vi "UI_Render_Main.vi"(0 "Channels":T1(array[cluster]), 1 "Logging":bool, 2 "Hover Button":i32=-1, 3 "Phase":bool, 5 "Data":dbl[][](array[numeric]), 7 "dt":dbl=0.001, 9 "Running":bool, 11 "error in":errorcluster, 12 "Status":string) -> (4 "Picture":picture, 15 "error out":errorcluster)   [LabVIEW 2026]
doc: "메인 화면 1600x940 전체 그리기: 주황 제목 띠 + 버튼 6개, 128채널 타일 바둑판, 하단 그래프 카드."
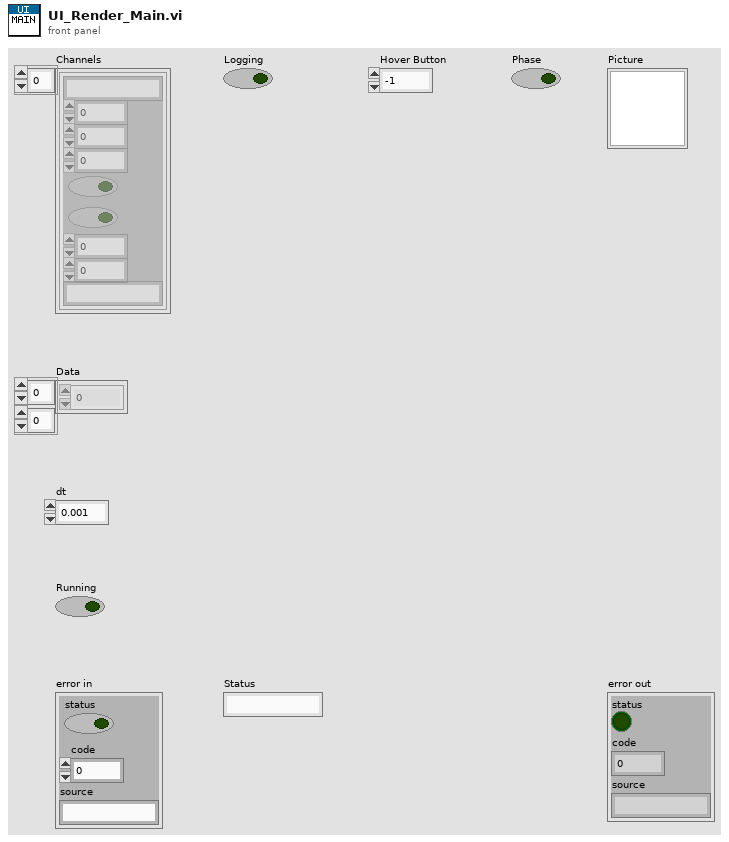
[diagram p1: front panel]
types:
  T1 = cluster{"Name":string, "Value":dbl, "High Limit":dbl, "Low Limit":dbl, "Save":bool, "Graph":bool, "Scale Min":dbl, "Scale Max":dbl, "Unit":string}[]
  T2 = cluster{"left":i16, "top":i16, "right":i16, "bottom":i16}
  T3 = cluster{"Font Name:":string, "Size":i16, "Strikeout?":bool, "Italic?":bool, "Underline?":bool, "Outline?":bool, "Shadow?":bool, "Bold?":bool}
  T4 = enum16{"User-specified Font", "Application Font", "System Font", "Dialog Font"}
  T5 = cluster{"horizontal":enum16{"left", "center", "right"}, "vertical":enum16{"top", "center", "bottom"}}
  T6 = cluster{"Width":u16, "Style":enum32{"Solid", "Dash", "Dot", "DashDot", "DashDotDot"}}
  T7 = cluster{"Rect":cluster{"left":i16, "top":i16, "right":i16, "bottom":i16}, "Fill":u32, "Fill Sel":u32, "Border":u32, "Border Sel":u32, "Text":string, "Text Color":u32, "Text Sel":u32, "Size":i16, "Bold":bool, "Group":i32, "Value":i32, "Radius":i16}[]
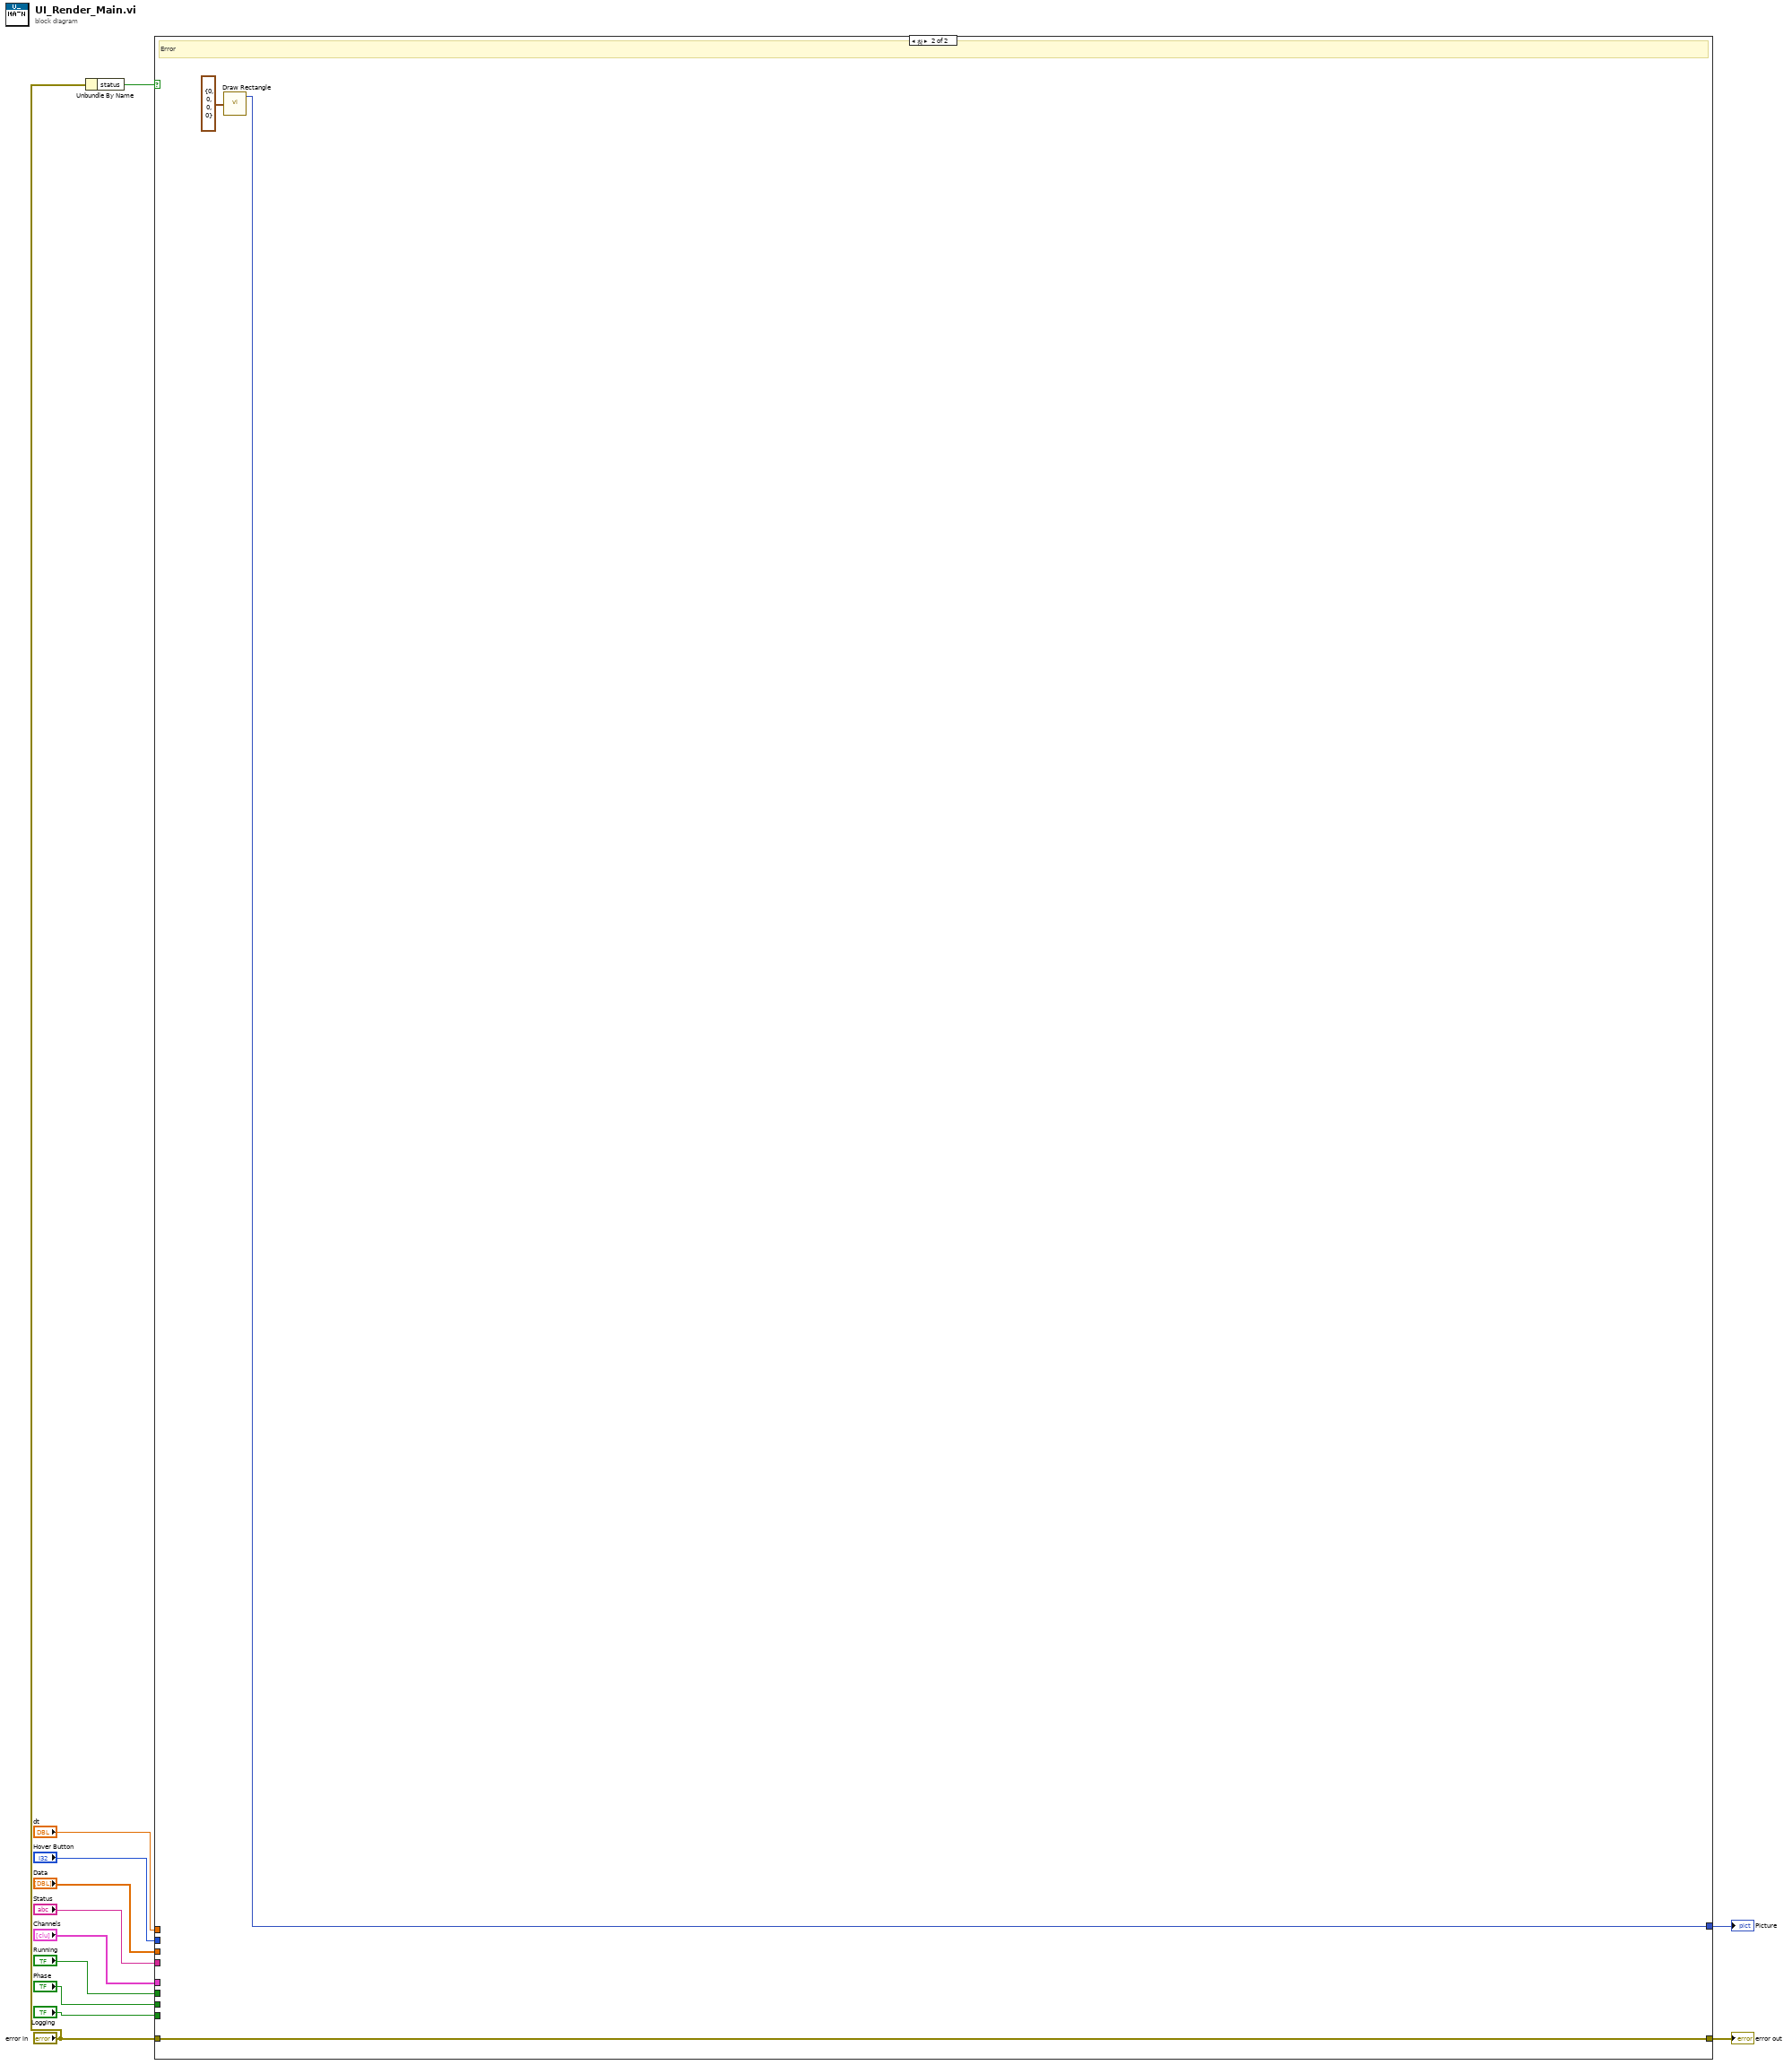
[diagram p0: block diagram]
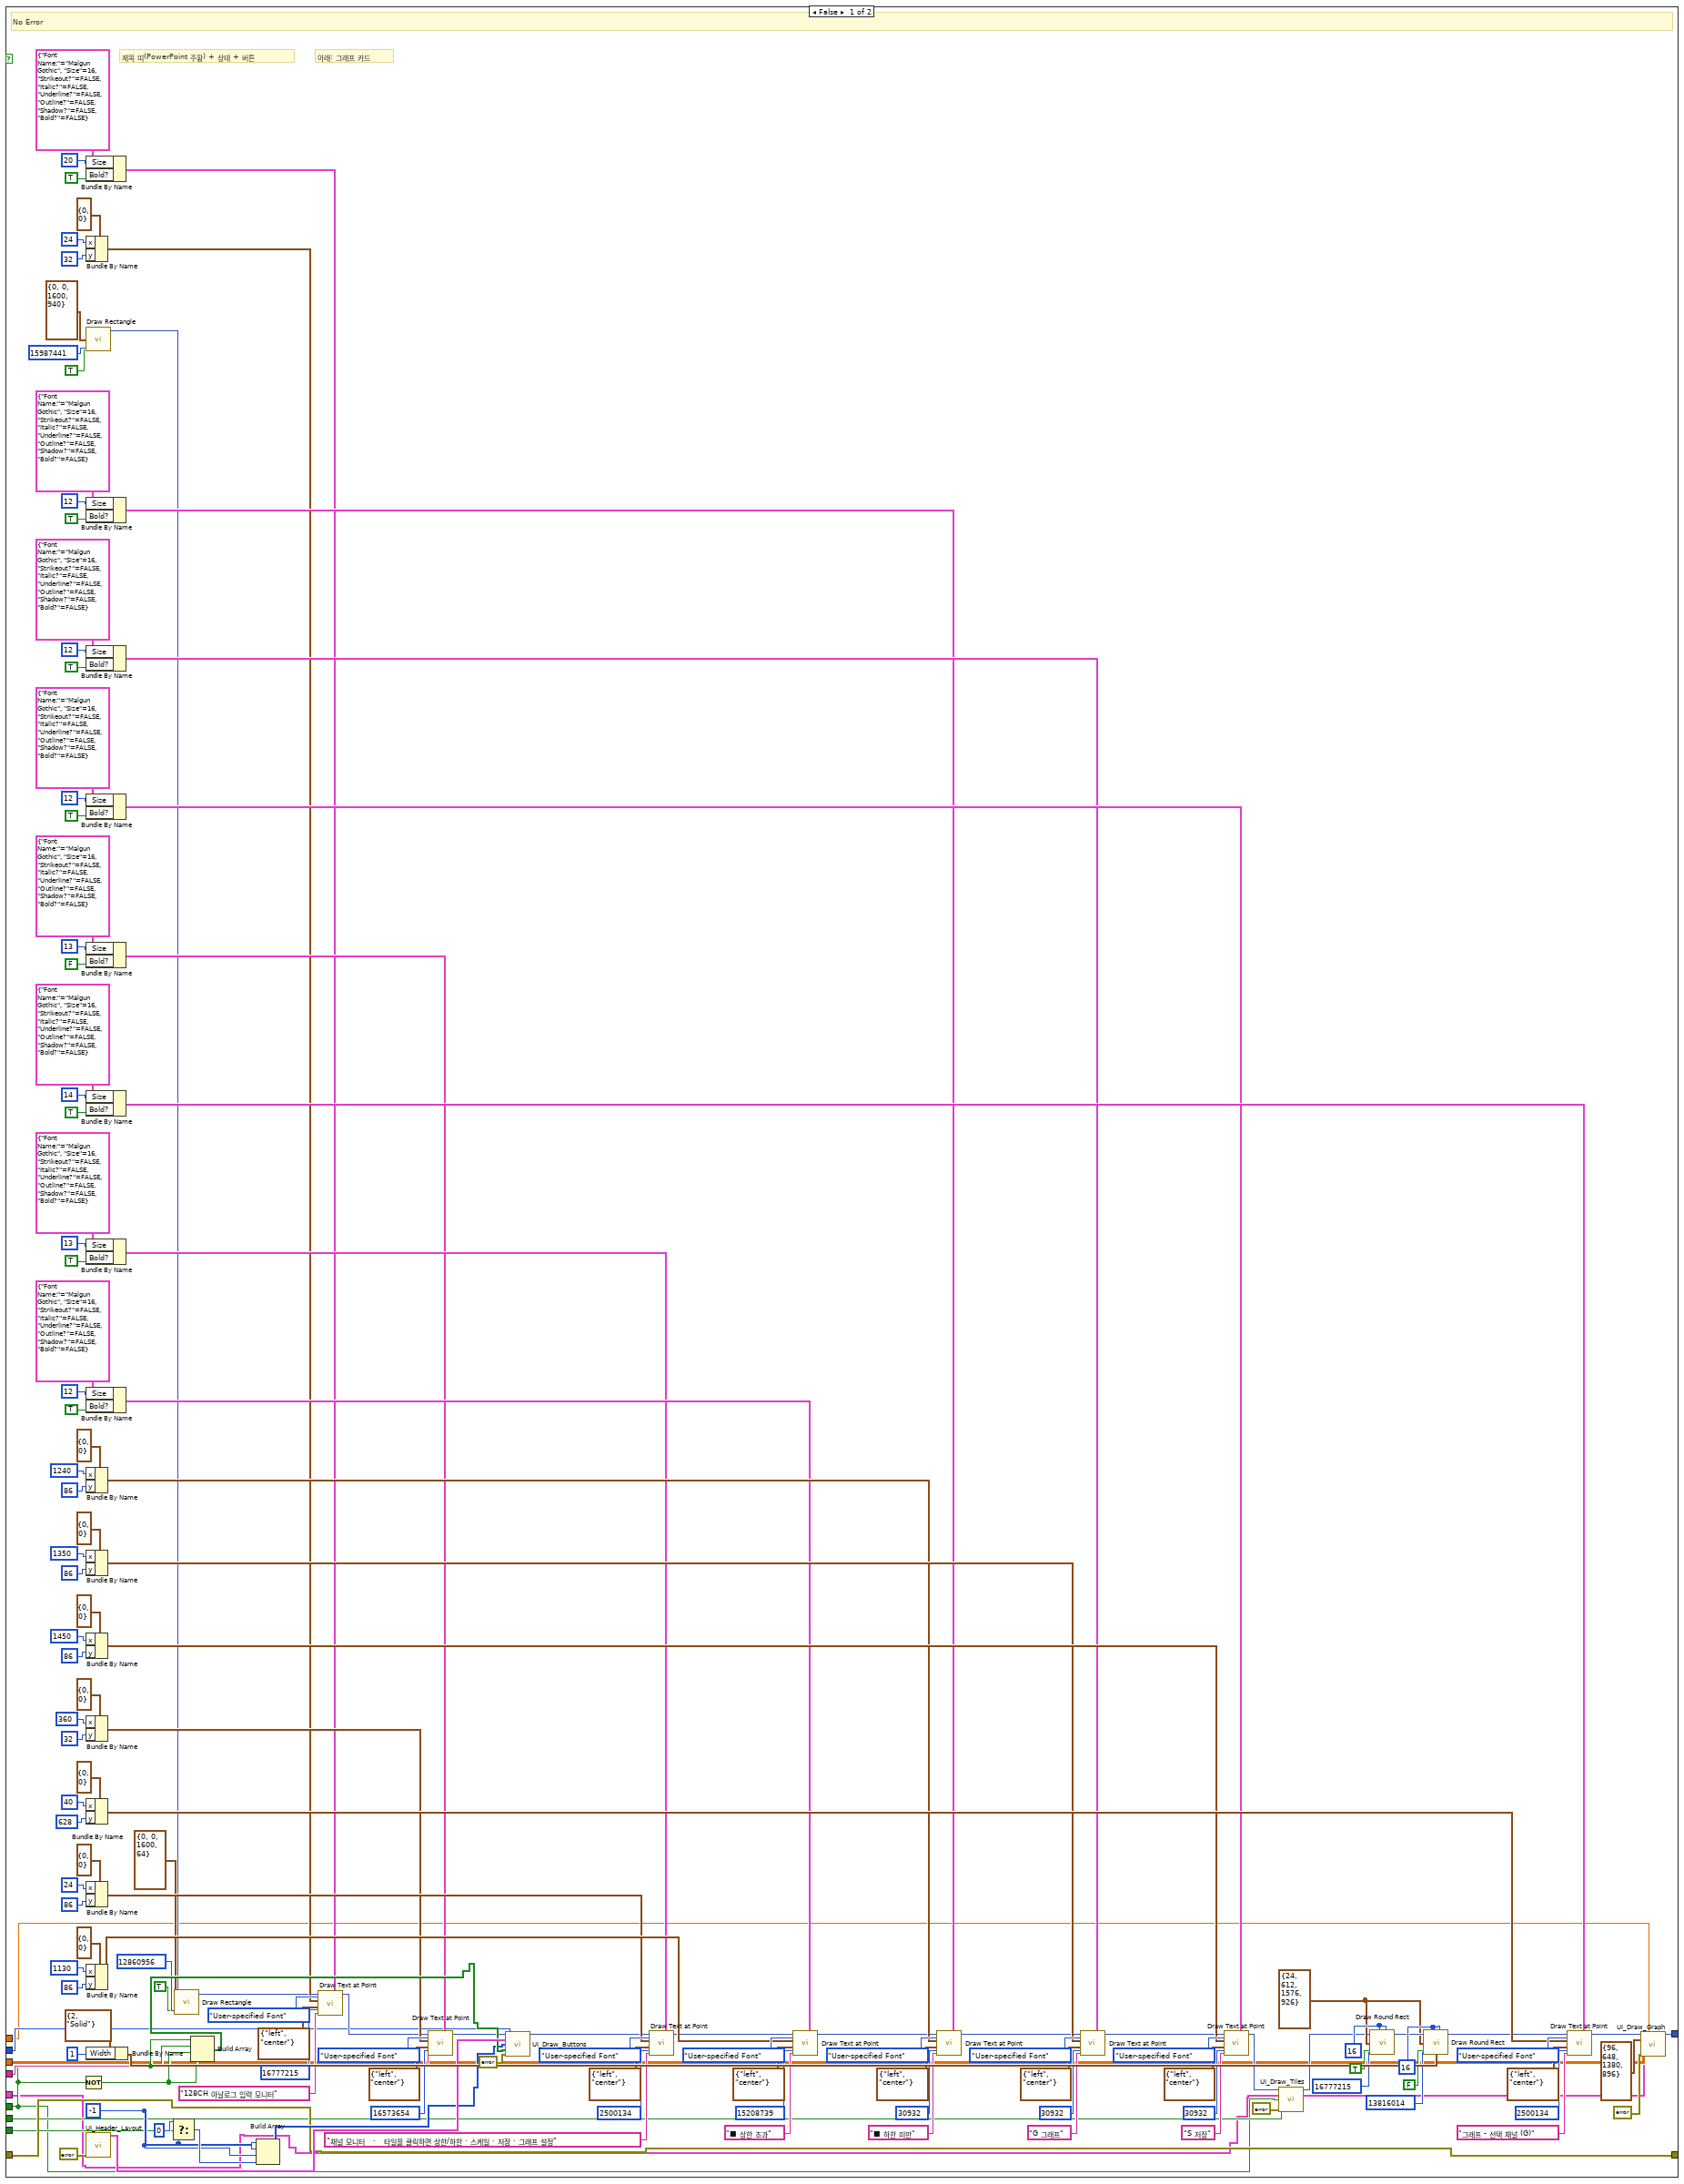
[diagram p2: hidden frame]
diagram:
  n1 = Unbundle By Name("error in") -> ("status"=w10:bool)
  n2 = case shown="참" w10 {
    tunnel: "Channels" -> [w13 _]
    tunnel: "Data" -> [w14 _]
    tunnel: "dt" -> [w15 _]
    tunnel: "Running" -> [w16 _]
    tunnel: "Logging" -> [w17 _]
    tunnel: "Hover Button" -> [w18 _]
    tunnel: "Phase" -> [w19 _]
    tunnel: "Status" -> [w20 _]
    tunnel: "error in" -> [w21 w160]
    tunnel: [w21 w160] -> w12
    tunnel: [w159 w162] -> w11
    frame False {
      w138 = i16 16
      w134 = i16 16
      w132 = T2 {"left"=24, "top"=612, "right"=1576, "bottom"=926}
      w55 = -1
      # "아래: 그래프 카드"
      # "제목 띠(PowerPoint 주황) + 상태 + 버튼"
      # "No Error"
      n3 = Not(x=w16) -> (.not. x?=w59:bool)
      n4 = Bundle By Name(cluster=T3 {"Font Name:"="Malgun Gothic", "Size"=16, "Strikeout?"=FALSE, "Italic?"=FALSE, "Underline?"=FALSE, "Outline?"=FALSE, "Shadow?"=FALSE, "Bold?"=FALSE}, "Size"=i16 20, "Bold?"=TRUE) -> (w41:T3)
      n5 = Bundle By Name(cluster=cluster{"x":i16, "y":i16} {"x"=0, "y"=0}, "x"=i16 24, "y"=i16 32) -> (w37:cluster{"x":i16, "y":i16})
      n6 = call <vilib>:"Draw Rectangle.vi"("rect"=T2 {"left"=0, "top"=0, "right"=1600, "bottom"=940}, "fill?(F)"=TRUE, "color(black)"=u32 15987441) -> ("new picture"=w25:picture)  [unwired: 6 in]
      n7 = Bundle By Name(cluster=T3 {"Font Name:"="Malgun Gothic", "Size"=16, "Strikeout?"=FALSE, "Italic?"=FALSE, "Underline?"=FALSE, "Outline?"=FALSE, "Shadow?"=FALSE, "Bold?"=FALSE}, "Size"=i16 12, "Bold?"=TRUE) -> (w102:T3)
      n8 = Bundle By Name(cluster=T3 {"Font Name:"="Malgun Gothic", "Size"=16, "Strikeout?"=FALSE, "Italic?"=FALSE, "Underline?"=FALSE, "Outline?"=FALSE, "Shadow?"=FALSE, "Bold?"=FALSE}, "Size"=i16 12, "Bold?"=TRUE) -> (w115:T3)
      n9 = Bundle By Name(cluster=T3 {"Font Name:"="Malgun Gothic", "Size"=16, "Strikeout?"=FALSE, "Italic?"=FALSE, "Underline?"=FALSE, "Outline?"=FALSE, "Shadow?"=FALSE, "Bold?"=FALSE}, "Size"=i16 12, "Bold?"=TRUE) -> (w128:T3)
      n10 = Bundle By Name(cluster=T3 {"Font Name:"="Malgun Gothic", "Size"=16, "Strikeout?"=FALSE, "Italic?"=FALSE, "Underline?"=FALSE, "Outline?"=FALSE, "Shadow?"=FALSE, "Bold?"=FALSE}, "Size"=i16 13, "Bold?"=FALSE) -> (w53:T3)
      n11 = Bundle By Name(cluster=T3 {"Font Name:"="Malgun Gothic", "Size"=16, "Strikeout?"=FALSE, "Italic?"=FALSE, "Underline?"=FALSE, "Outline?"=FALSE, "Shadow?"=FALSE, "Bold?"=FALSE}, "Size"=i16 14, "Bold?"=TRUE) -> (w155:T3)
      n12 = Bundle By Name(cluster=T3 {"Font Name:"="Malgun Gothic", "Size"=16, "Strikeout?"=FALSE, "Italic?"=FALSE, "Underline?"=FALSE, "Outline?"=FALSE, "Shadow?"=FALSE, "Bold?"=FALSE}, "Size"=i16 13, "Bold?"=TRUE) -> (w76:T3)
      n13 = Bundle By Name(cluster=T3 {"Font Name:"="Malgun Gothic", "Size"=16, "Strikeout?"=FALSE, "Italic?"=FALSE, "Underline?"=FALSE, "Outline?"=FALSE, "Shadow?"=FALSE, "Bold?"=FALSE}, "Size"=i16 12, "Bold?"=TRUE) -> (w89:T3)
      n14 = Bundle By Name(cluster=cluster{"x":i16, "y":i16} {"x"=0, "y"=0}, "x"=i16 1240, "y"=i16 86) -> (w98:cluster{"x":i16, "y":i16})
      n15 = Bundle By Name(cluster=cluster{"x":i16, "y":i16} {"x"=0, "y"=0}, "x"=i16 1350, "y"=i16 86) -> (w111:cluster{"x":i16, "y":i16})
      n16 = Bundle By Name(cluster=cluster{"x":i16, "y":i16} {"x"=0, "y"=0}, "x"=i16 1450, "y"=i16 86) -> (w124:cluster{"x":i16, "y":i16})
      n17 = Bundle By Name(cluster=cluster{"x":i16, "y":i16} {"x"=0, "y"=0}, "x"=i16 360, "y"=i16 32) -> (w49:cluster{"x":i16, "y":i16})
      n18 = Bundle By Name(cluster=cluster{"x":i16, "y":i16} {"x"=0, "y"=0}, "x"=i16 40, "y"=i16 628) -> (w151:cluster{"x":i16, "y":i16})
      n19 = Bundle By Name(cluster=cluster{"x":i16, "y":i16} {"x"=0, "y"=0}, "x"=i16 24, "y"=i16 86) -> (w72:cluster{"x":i16, "y":i16})
      n20 = Bundle By Name(cluster=cluster{"x":i16, "y":i16} {"x"=0, "y"=0}, "x"=i16 1130, "y"=i16 86) -> (w85:cluster{"x":i16, "y":i16})
      n21 = Bundle By Name(cluster=T6 {"Width"=2, "Style"=enum."Solid"}, "Width"=u16 1) -> (w142:T6)
      n22 = call "UI_Header_Layout.vi"("error in"=errorcluster {"status"=FALSE, "code"=0, "source"=""}) -> ("Specs"=w62:T7)  [unwired: 13 in, 1 out]
      n23 = Select(t=0, s=w17, f=w55) -> (s? t:f=w57:i32)
      n24 = call <vilib>:"Draw Rectangle.vi"("picture"=w25, "rect"=T2 {"left"=0, "top"=0, "right"=1600, "bottom"=64}, "fill?(F)"=TRUE, "color(black)"=u32 12860956) -> ("new picture"=w29:picture)  [unwired: 5 in]
      n25 = Build Array(w16, w16, w59, w59) -> (w60:bool[])
      n26 = Build Array(w55, w55, w55, w57) -> (w58:i32[])
      n27 = call <vilib>:"Draw Text at Point.vi"("[user-specified font]"=w41, "text color(black)"=u32 16777215, "desired font(Application)"=T4."User-specified Font", "text"="128CH 아날로그 입력 모니터", "alignment(left, top)"=T5 {"horizontal"=enum."left", "vertical"=enum."center"}, "origin"=w37, "picture"=w29) -> ("new picture"=w42:picture)  [unwired: 3 in, 1 out]
      n28 = call <vilib>:"Draw Text at Point.vi"("[user-specified font]"=w53, "text color(black)"=u32 16573654, "desired font(Application)"=T4."User-specified Font", "text"=w20, "alignment(left, top)"=T5 {"horizontal"=enum."left", "vertical"=enum."center"}, "origin"=w49, "picture"=w42) -> ("new picture"=w54:picture)  [unwired: 3 in, 1 out]
      n29 = call "UI_Draw_Buttons.vi"("Picture"=w54, "Hover"=w18, "Specs"=w62, "Values"=w58, "Dim Groups"=w60, "error in"=errorcluster {"status"=FALSE, "code"=0, "source"=""}) -> ("New Picture"=w64:picture)  [unwired: 8 in, 1 out]
      n30 = call <vilib>:"Draw Text at Point.vi"("[user-specified font]"=w76, "text color(black)"=u32 2500134, "desired font(Application)"=T4."User-specified Font", "text"="채널 모니터   ·   타일을 클릭하면 상한/하한 · 스케일 · 저장 · 그래프 설정", "alignment(left, top)"=T5 {"horizontal"=enum."left", "vertical"=enum."center"}, "origin"=w72, "picture"=w64) -> ("new picture"=w77:picture)  [unwired: 3 in, 1 out]
      n31 = call <vilib>:"Draw Text at Point.vi"("[user-specified font]"=w89, "text color(black)"=u32 15208739, "desired font(Application)"=T4."User-specified Font", "text"="■ 상한 초과", "alignment(left, top)"=T5 {"horizontal"=enum."left", "vertical"=enum."center"}, "origin"=w85, "picture"=w77) -> ("new picture"=w90:picture)  [unwired: 3 in, 1 out]
      n32 = call <vilib>:"Draw Text at Point.vi"("[user-specified font]"=w102, "text color(black)"=u32 30932, "desired font(Application)"=T4."User-specified Font", "text"="■ 하한 미만", "alignment(left, top)"=T5 {"horizontal"=enum."left", "vertical"=enum."center"}, "origin"=w98, "picture"=w90) -> ("new picture"=w103:picture)  [unwired: 3 in, 1 out]
      n33 = call <vilib>:"Draw Text at Point.vi"("[user-specified font]"=w115, "text color(black)"=u32 30932, "desired font(Application)"=T4."User-specified Font", "text"="G 그래프", "alignment(left, top)"=T5 {"horizontal"=enum."left", "vertical"=enum."center"}, "origin"=w111, "picture"=w103) -> ("new picture"=w116:picture)  [unwired: 3 in, 1 out]
      n34 = call <vilib>:"Draw Text at Point.vi"("[user-specified font]"=w128, "text color(black)"=u32 30932, "desired font(Application)"=T4."User-specified Font", "text"="S 저장", "alignment(left, top)"=T5 {"horizontal"=enum."left", "vertical"=enum."center"}, "origin"=w124, "picture"=w116) -> ("new picture"=w129:picture)  [unwired: 3 in, 1 out]
      n35 = call "UI_Draw_Tiles.vi"("Picture"=w129, "Channels"=w13, "Running"=w16, "Phase"=w19, "error in"=errorcluster {"status"=FALSE, "code"=0, "source"=""}) -> ("New Picture"=w131:picture)  [unwired: 9 in, 1 out]
      n36 = call <vilib>:"Draw Round Rect.vi"("picture"=w131, "oval width"=w134, "rect"=w132, "fill?(F)"=TRUE, "color(black)"=u32 16777215, "oval height"=w134) -> ("new picture"=w136:picture)  [unwired: 3 in]
      n37 = call <vilib>:"Draw Round Rect.vi"("picture"=w136, "oval width"=w138, "rect"=w132, "fill?(F)"=FALSE, "color(black)"=u32 13816014, "oval height"=w138, "pen"=w142) -> ("new picture"=w143:picture)  [unwired: 2 in]
      n38 = call <vilib>:"Draw Text at Point.vi"("[user-specified font]"=w155, "text color(black)"=u32 2500134, "desired font(Application)"=T4."User-specified Font", "text"="그래프 - 선택 채널 (G)", "alignment(left, top)"=T5 {"horizontal"=enum."left", "vertical"=enum."center"}, "origin"=w151, "picture"=w143) -> ("new picture"=w156:picture)  [unwired: 3 in, 1 out]
      n39 = call "UI_Draw_Graph.vi"("Picture"=w156, "dt"=w15, "Plot Rect"=T2 {"left"=96, "top"=648, "right"=1380, "bottom"=896}, "Data"=w14, "Channels"=w13, "error in"=errorcluster {"status"=FALSE, "code"=0, "source"=""}) -> ("New Picture"=w159:picture)  [unwired: 8 in, 1 out]
    }
    frame True {
      # "Error"
      n40 = call <vilib>:"Draw Rectangle.vi"("rect"=T2 {"left"=0, "top"=0, "right"=0, "bottom"=0}) -> ("new picture"=w162:picture)  [unwired: 8 in]
    }
  }
  "Picture" <- w11
  "error out" <- w12
